vi "Add Client to Service.vi"(8 "error in (no error)":errorcluster, 9 "Client ID":string, 10 "WebSocket Connection in":refnum<k5>, 11 "WebSocket Server in":refnum<class "WebSocket Server.lvclass">) -> (0 "error out":errorcluster, 3 "WebSocket Server out":refnum<class "WebSocket Server.lvclass">)   [LabVIEW 2021, in "WebSocket Actors.lvlib" / "WebSocket Server.lvclass"]
doc: "This method performs the WebSocket handshake upon an incoming connection. If the service requested is defined in this server, we send a message to the corresponding service to add the client to its clients list. If either the service is not defined, or the handshake fails we do nothing, the WebSocket protocol will take care of communicating the failure to the client."
uses:
  WebSocket Server.lvclass
  WebSocket Server.lvclass/WebSocket Server.ctl
  <vilib>/GPower/Error/Library/SplitAppended.vi
  <vilib>/GPower/Error/Library/AppendErrors.vi
  <vilib>/GPower/Error/Library/Append/AppendMulti.vi
  <vilib>/GPower/Error/Library/SubVIs/ExplanationToError.vi
  <vilib>/dlg_ctls.llb/Space Constant.vi
  <vilib>/Utility/error.llb/Trim Whitespace.vi
  <vilib>/Utility/error.llb/Error Code Database.vi
  <vilib>/GPower/Error/Library/Append/AppendSingle.vi
  WebSocket Service Messages/Add Client Msg/Add Client Msg.lvclass
  <vilib>/GPower/Error/GPError.lvlib
  <vilib>/LS Instruments AG/LV-WebSockets/LV WebSockets.lvlib
panel:
  out "Resource Name":string
  out "HTTP Headers":variant
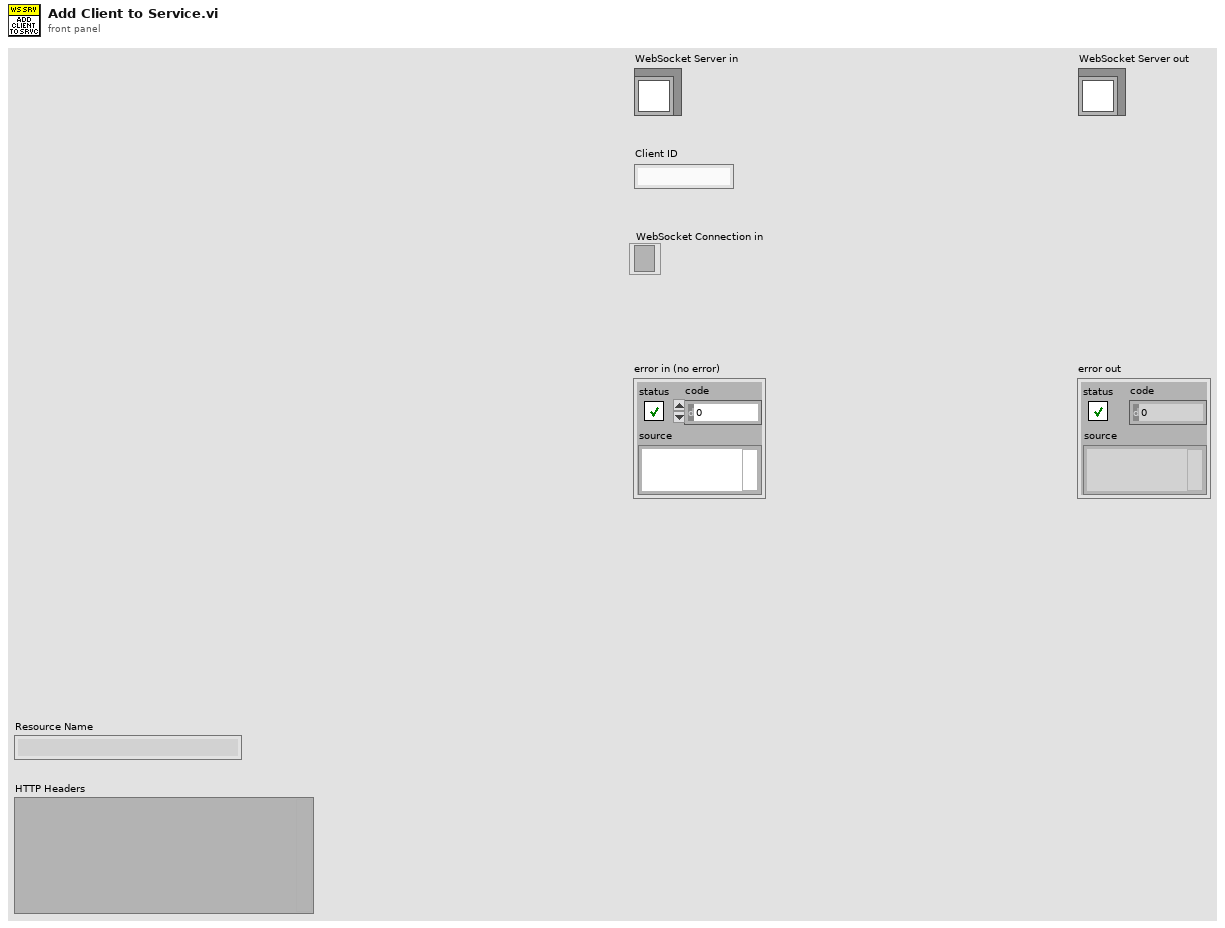
[diagram p1: front panel]
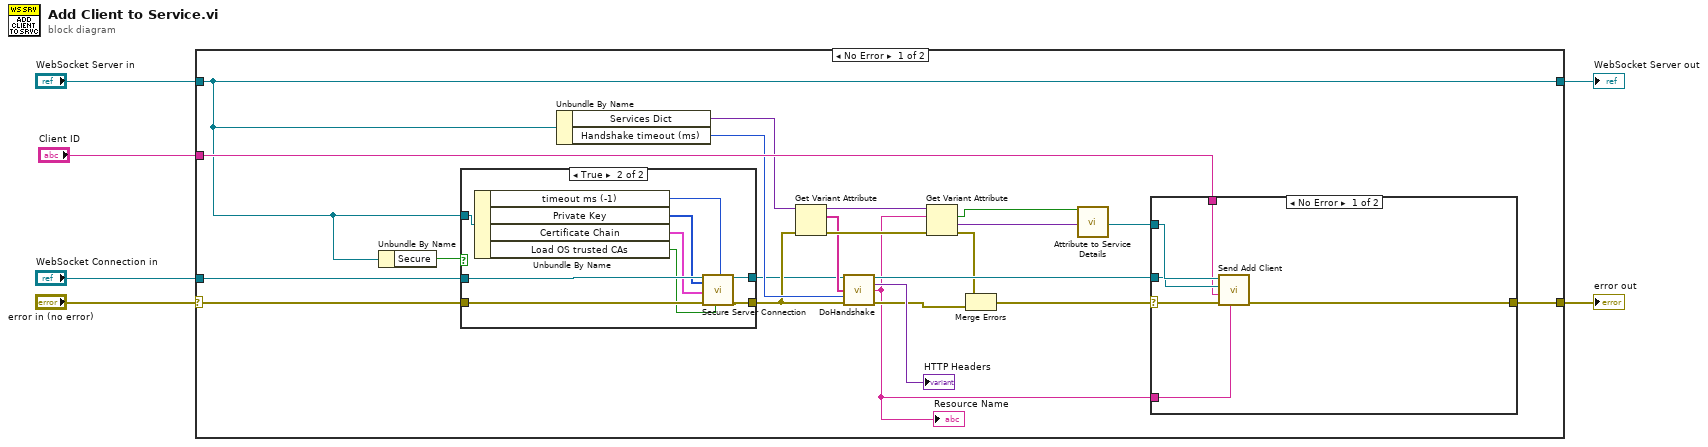
[diagram p0: block diagram]
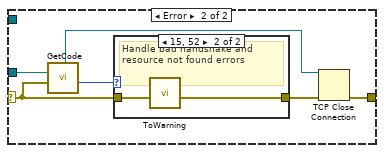
[diagram p3: hidden frame]
diagram:
  n1 = case shown="No Error" "error in (no error)" {
    selector: "error in (no error)" -> [w11 w55]
    tunnel: [w20 w55] -> w5
    tunnel: [w8 w54] -> w3
    tunnel: "WebSocket Server in" -> [w8 w54]
    tunnel: "WebSocket Connection in" -> [w10 _]
    tunnel: "Client ID" -> [w19 _]
    frame No Error {
      n2 = Unbundle By Name(w8) -> ("Secure"=w7:bool)
      n3 = case shown="True" w7 {
        tunnel: [w30 w39] -> w12
        tunnel: w11 -> [w30 w38]
        tunnel: w10 -> [w29 w37]
        tunnel: [w29 w36] -> w9
        tunnel: w8 -> [_ w35]
        frame False {
        }
        frame True {
          n4 = Unbundle By Name(w35) -> ("timeout ms (-1)"=w34:i32, "Private Key"=w33:u8[], "Certificate Chain"=w32:cluster{"certificate":u8[]}[], "Load OS trusted CAs"=w31:bool)
          n5 = call <vilib>:"Secure Server Connection.vi"("TCP connection"=w37, "private key"=w33, "certificate chain"=w32, "error in"=w38, "load OS trusted CAs?"=w31, "timeout (25000 ms)"=w34) -> ("TCP connection out"=w36:refnum<k5>, "error out"=w39:errorcluster)  [unwired: 11 in, 1 out]
        }
      }
      n6 = Unbundle By Name(w8) -> ("Services Dict"=w17:variant, "Handshake timeout (ms)"=w18:i32)
      n7 = Get Variant Attribute(Variant=w17, error in=w12) -> (duplicate Variant=w15:variant, names=w14:string[], error out=w16:errorcluster)  [unwired: 2 in, 1 out]
      n8 = call <vilib>:"DoHandshake.vi"("WebSocket Connection in"=w9, "Resource Names"=w14, "timeout ms (5000)"=w18, "error in (no error)"=w12) -> ("WebSocket Connection out"=w27:refnum<k5>, "Headers Out"=→"HTTP Headers":variant, "Resource Name"=w13:string, "error out"=w25:errorcluster)  [unwired: 6 in, 2 out]
      "Resource Name" <- w13
      n9 = Get Variant Attribute(Variant=w15, name=w13, error in=w16) -> (found=w23:bool, value=w22:variant, error out=w24:errorcluster)  [unwired: 1 in, 1 out]
      n10 = Merge Errors(w24, w25) -> (w26:errorcluster)
      n11 = call "Attribute to Service Details.vi"("Attibute Found"=w23, "Attribute"=w22) -> ("Service Enqueuer"=w21:refnum<class "Message Enqueuer.lvclass">)  [unwired: 17 in]
      n12 = case shown="No Error" w26 {
        selector: w26 -> [w45 w47]
        tunnel: w27 -> [w42 w49]
        tunnel: [w44 w50] -> w20
        tunnel: w21 -> [w43 _]
        tunnel: w19 -> [w41 _]
        tunnel: w13 -> [w40 _]
        frame No Error {
          n13 = call "Send Add Client.vi"("Service Name"=w40, "error in (no error)"=w45, "Client ID"=w41, "WebSocket Connection"=w42, "Message Enqueuer in"=w43) -> ("error out"=w44:errorcluster)  [unwired: 5 in, 1 out]
        }
        frame Error {
          n14 = call <vilib>:"GetCode.vi"("Error in"=w47) -> ("Code"=w48:i32)  [unwired: 10 in]
          n15 = case shown="15, 52" w48 {
            tunnel: w47 -> [w51 w53]
            tunnel: [w51 w52] -> w46
            frame 0, Default {
              # "Unknown error"
            }
            frame 15, 52 {
              # "Handle bad handshake and resource not found errors"
              n16 = call <vilib>:"ToWarning.vi"("Error in"=w53) -> ("Warning out"=w52:errorcluster)  [unwired: 10 in]
            }
          }
          n17 = TCP Close Connection(connection ID=w49, error in (no error)=w46) -> (error out=w50:errorcluster)  [unwired: 1 in, 1 out]
        }
      }
    }
    frame Error {
    }
  }
  "error out" <- w5
  "WebSocket Server out" <- w3
